vi "Execute.vi"(8 "error in (no error)":errorcluster, 11 "CIFPlugin in":refnum<class "CAN_Writer_CANsub_Plugin.lvclass">) -> (0 "error out":errorcluster, 3 "CIFPlugin out":refnum<class "CAN_Writer_CANsub_Plugin.lvclass">)   [LabVIEW 2021, in "CAN_Writer_CANsub_Plugin.lvclass"]
uses:
  CAN_Writer_CANsub_Plugin.lvclass
  CAN_Writer_CANsub_Plugin.lvclass/CAN_Writer_CANsub_Plugin.ctl
  <vilib>/CIF Foundation/CIF Core/CIFCore/Class/Typedef/Energized States.ctl
  <vilib>/CIF Foundation/CIF Core/CIFCore/Class/CIFCorePlugin.lvclass
  C:/Program Files/National Instruments/LabVIEW 2021/vi.lib/CIF Foundation/CIF Core/CIFCore/Class/CIFCorePlugin.lvclass
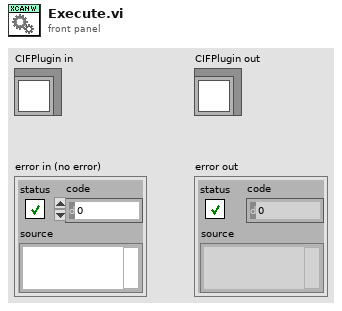
[diagram p1: front panel]
types:
  T1 = typedef "CIFCorePlugin.lvclass/Energized States.ctl" = enum8{"Listen", "Prepare", "Execute", "Housekeep", "Cleanup", "Destroy"}
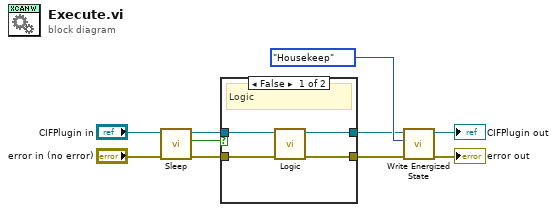
[diagram p0: block diagram]
diagram:
  n1 = call <vilib>:"Sleep.vi"("error in (no error)"="error in (no error)", "CIFCorePlugin in"="CIFPlugin in") -> ("error out"=w7:errorcluster, "Housekeep only"=w8:bool, "CIFCorePlugin out"=w6:refnum<class "CAN_Writer_CANsub_Plugin.lvclass">)  [unwired: 7 in]
  n2 = case shown="False" w8 {
    tunnel: [w12 w15] -> w1
    tunnel: [w13 w16] -> w9
    tunnel: w6 -> [w14 w16]
    tunnel: w7 -> [w11 w15]
    frame False {
      # "Logic"
      n3 = call "Logic.vi"("error in (no error)"=w11, "CIFPlugin in"=w14) -> ("error out"=w12:errorcluster, "CIFPlugin out"=w13:refnum<class "CAN_Writer_CANsub_Plugin.lvclass">)  [unwired: 8 in]
    }
    frame True {
      # "Housekeep only"
    }
  }
  n4 = call <vilib>:"Write Energized State.vi"("error in (no error)"=w1, "Energized State"=Energized_States."Housekeep", "CIFCorePlugin in"=w9) -> ("error out"=→"error out":errorcluster, "CIFCorePlugin in"=→"CIFPlugin out":refnum<class "CAN_Writer_CANsub_Plugin.lvclass">)  [unwired: 7 in]
